vi "Move Clock Wise.vi"(8 "error in (no error)":errorcluster, 11 "ETS_EM2090 in":refnum<class "ETS_EM2090.lvclass">) -> (0 "error out":errorcluster, 3 "ETS_EM2090 out":refnum<class "ETS_EM2090.lvclass">)   [LabVIEW 2023, in "Turn Table and Mast.lvlib" / "ETS_EM2090.lvclass"]
uses:
  ETS_EM2090.lvclass
  ETS_EM2090.lvclass/ETS_EM2090.ctl
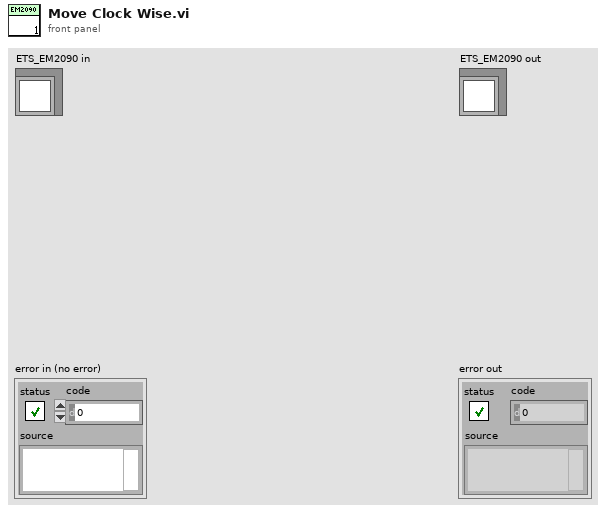
[diagram p1: front panel]
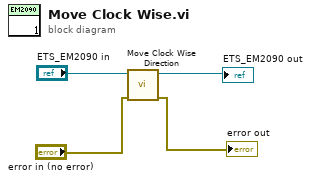
[diagram p0: block diagram]
diagram:
  n1 = call "Move Clock Wise Direction.vi"("error in (no error)"="error in (no error)", "ETS_EM2090 in"="ETS_EM2090 in") -> ("error out"=→"error out":errorcluster, "ETS_EM2090 out"=→"ETS_EM2090 out":refnum<class "ETS_EM2090.lvclass">)  [unwired: 8 in]
